vi "login credentials FG.vi"(6 "FG action":T1, 8 "error in":errorcluster, 11 "device class":T3={"cDAQ"=TRUE, "cRIO"=TRUE, "Ethernet RIO"=TRUE, "sbRIO"=TRUE, "PXI"=FALSE, "CVS"=FALSE, "Desktop"=FALSE, "FieldPoint"=FALSE, "<No Device Class>"=FALSE}) -> (0 "error out":errorcluster, 3 "login credentials":T2[](array[typedef]))   [LabVIEW 2014, in "tests.lvlib"]
uses:
  tests.lvlib
  classes/Device/device class selection.ctl
  classes/Device/login credentials.ctl
  classes/Device/FG action.ctl
  classes/Device/device login credentials.ctl
  classes/Device/device class.ctl
  <vilib>/regexp/Match Regular Expression.xnode
  classes/Device/Device.lvclass
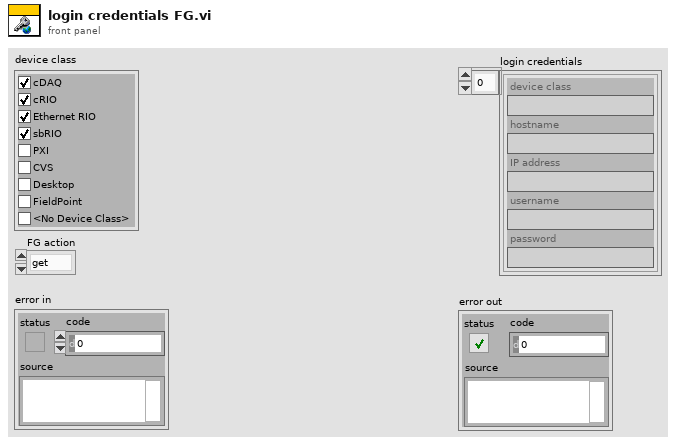
[diagram p1: front panel]
types:
  T1 = typedef "SMI.lvlib/Device.lvclass/FG action.ctl" = enum16{"get", "set"}
  T2 = typedef "SMI.lvlib/Device.lvclass/login credentials.ctl" = cluster{"device class":string, "hostname":string, "IP address":string, "username":string, "password":string}
  T3 = typedef "SMI.lvlib/Device.lvclass/device class selection.ctl" = cluster{"cDAQ":bool, "cRIO":bool, "Ethernet RIO":bool, "sbRIO":bool, "PXI":bool, "CVS":bool, "Desktop":bool, "FieldPoint":bool, "<No Device Class>":bool}
  T4 = typedef "SMI.lvlib/Device.lvclass/device login credentials.ctl" = cluster{"device class":T5, "hostname regular expression":string, "username":string, "password":string}
  T5 = typedef "SMI.lvlib/Device.lvclass/device class.ctl" = enum16{"cDAQ", "cRIO", "Ethernet RIO", "sbRIO", "PXI", "CVS", "Desktop", "FieldPoint", "<No Device Class>", "<Detect All>"}
  T6 = typedef "SMI.lvlib/Device.lvclass/network device information.ctl" = cluster{"hostname":string, "IP address":string, "MAC address":string, "vendor name":string, "product name":string, "product ID":u16, "serial number":string, "device class":string}
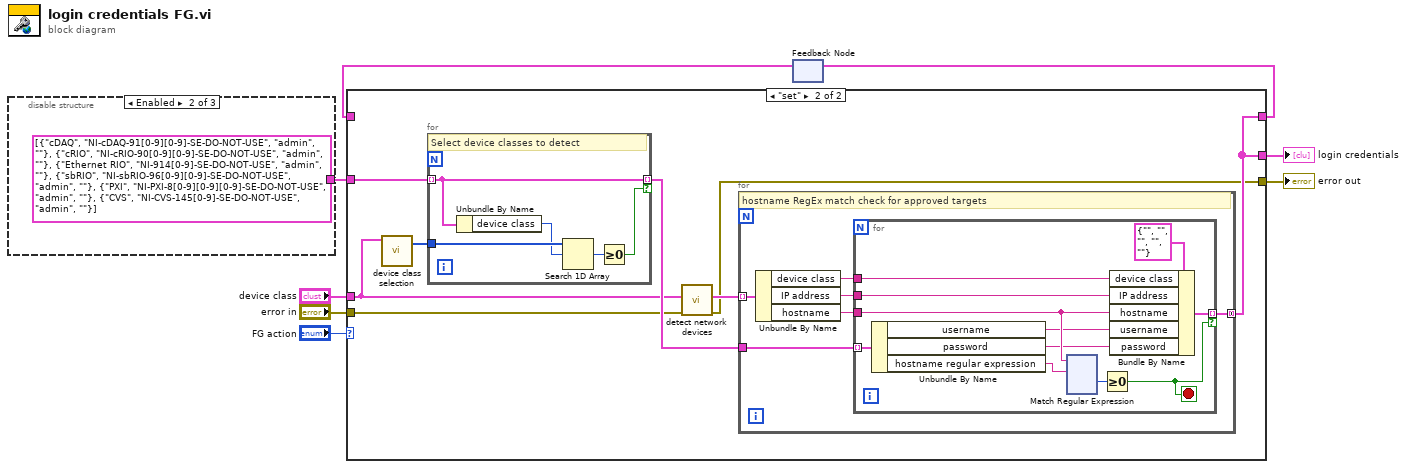
[diagram p0: block diagram]
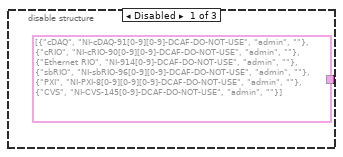
[diagram p2: hidden frame]
diagram:
  n1 = disable-structure shown="Enabled" {
    disable-tunnel: [T4[] [{"device class"=enum."cDAQ", "hostname regular expression"="NI-cDAQ-91[0-9][0-9]-DCAF-DO-NOT-USE", "username"="admin", "password"=""}, {"device class"=enum."cRIO", "hostname regular expression"="NI-cRIO-90[0-9][0-9]-DCAF-DO-NOT-USE", "username"="admin", "password"=""}, {"device class"=enum."Ethernet RIO", "hostname regular expression"="NI-914[0-9]-DCAF-DO-NOT-USE", "username"="admin", "password"=""}, {"device class"=enum."sbRIO", "hostname regular expression"="NI-sbRIO-96[0-9][0-9]-DCAF-DO-NOT-USE", "username"="admin", "password"=""}, {"device class"=enum."PXI", "hostname regular expression"="NI-PXI-8[0-9][0-9][0-9]-DCAF-DO-NOT-USE", "username"="admin", "password"=""}, {"device class"=enum."CVS", "hostname regular expression"="NI-CVS-145[0-9]-DCAF-DO-NOT-USE", "username"="admin", "password"=""}] T4[] [{"device class"=enum."cDAQ", "hostname regular expression"="NI-cDAQ-91[0-9][0-9]-SE-DO-NOT-USE", "username"="admin", "password"=""}, {"device class"=enum."cRIO", "hostname regular expression"="NI-cRIO-90[0-9][0-9]-SE-DO-NOT-USE", "username"="admin", "password"=""}, {"device class"=enum."Ethernet RIO", "hostname regular expression"="NI-914[0-9]-SE-DO-NOT-USE", "username"="admin", "password"=""}, {"device class"=enum."sbRIO", "hostname regular expression"="NI-sbRIO-96[0-9][0-9]-SE-DO-NOT-USE", "username"="admin", "password"=""}, {"device class"=enum."PXI", "hostname regular expression"="NI-PXI-8[0-9][0-9][0-9]-SE-DO-NOT-USE", "username"="admin", "password"=""}, {"device class"=enum."CVS", "hostname regular expression"="NI-CVS-145[0-9]-SE-DO-NOT-USE", "username"="admin", "password"=""}] _] -> w2
    frame Disabled {
    }
    frame Enabled {
    }
    frame Disabled {
    }
  }
  n2 = feedback #1() -> (w6:T2[])  [unwired: 1 in]
  n3 = case shown="\"set\"" "FG action" {
    tunnel: "device class" -> [_ w16]
    tunnel: [w12 w17] -> w7
    tunnel: w6 -> [w12 _]
    tunnel: [w12 w17] -> w5
    tunnel: [w11 w15] -> w3
    tunnel: "error in" -> [w11 w13]
    tunnel: w2 -> [_ w14]
    frame "get", Default {
    }
    frame "set" {
      n4 = call "device class selection.vi"("device classes"=w16) -> ("device class"=w20:T5[])  [unwired: 6 in]
      n5 = for {
        tunnel: [w152] -> w18 mode=indexing if=w154
        tunnel: w20 -> [w156]
        tunnel: w14 -> [w152] mode=indexing
        # "Select device classes to detect"
        n6 = Unbundle By Name(w152) -> ("device class"=w153:T5)
        n7 = Search 1D Array(1D array=w156, element=w153) -> (index of element=w155:i32)  [unwired: 1 in]
        n8 = Greater Or Equal To 0?(x=w155) -> (x >= 0?=w154:bool)
      }
      n9 = call "detect network devices.vi"("error in"=w13, "device class"=w16) -> ("error out"=w15:errorcluster, "devices"=w19:T6[])  [unwired: 7 in, 1 out]
      n10 = for {
        tunnel: w19 -> [w26] mode=indexing
        tunnel: w18 -> [w25]
        tunnel: [w23] -> w17 mode=concatenating
        # "hostname RegEx match check for approved targets"
        n11 = Unbundle By Name(w26) -> ("device class"=w21:string, "IP address"=w22:string, "hostname"=w24:string)
        n12 = for {
          tunnel: w25 -> [w36] mode=indexing
          tunnel: w24 -> [w31]
          tunnel: [w35] -> w23 mode=indexing if=w29
          tunnel: w22 -> [w33]
          tunnel: w21 -> [w32]
          stop <- w29 stop-if-true
          n13 = Unbundle By Name(w36) -> ("username"=w27:string, "password"=w28:string, "hostname regular expression"=w37:string)
          n14 = xnode "Match Regular Expression"("input string"=w31, "regular expression"=w37) -> ("offset past match"=w34:i32)  [unwired: 4 in, 4 out]
          n15 = Greater Or Equal To 0?(x=w34) -> (x >= 0?=w29:bool)
          n16 = Bundle By Name(cluster=T2 {"device class"="", "hostname"="", "IP address"="", "username"="", "password"=""} ("login credentials"), "device class"=w32, "IP address"=w33, "hostname"=w31, "username"=w27, "password"=w28) -> (w35:T2)
        }
      }
    }
  }
  "login credentials" <- w5
  "error out" <- w3
  n17 = feedback-in #1(w7) -> ()
